vi "test_DependencyList_FilterByMatchingString.vi"() -> (3 "Pass?":bool)   [LabVIEW 2020, in "Tests.DependencyInspection.lvlib"]
uses:
  Tests.DependencyInspection.lvlib
  CDependencyList/CDependencyList.lvclass
  ItemInfo.ctl
  CItemMatch/CItemMatch.lvclass
  CItemMatch/TypeDefs/Field.ctl
  CItemMatch/TypeDefs/ComparisonType.ctl
  CDependencyList/ListGenerationOptions.ctl
panel:
  out "Array":string[](array[string])
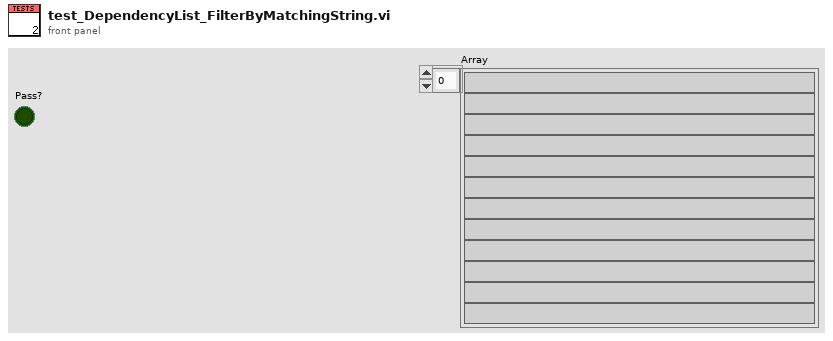
[diagram p1: front panel]
types:
  T1 = typedef "Tests.DependencyInspection.lvlib/ItemInfo.ctl" = cluster{"path":path, "delimited name":string}
  T2 = typedef "DependencyInspection.lvlib/CItemMatch.lvclass/ComparisonType.ctl" = enum16{"None", "Ends with", "Equals", "Not equal", "Starts with", "Contains", "Matches pattern"}
  T3 = typedef "DependencyInspection.lvlib/CItemMatch.lvclass/Field.ctl" = enum16{"Name", "Qualified name", "Path"}
  T4 = typedef "DependencyInspection.lvlib/CDependencyList.lvclass/ListGenerationOptions.ctl" = cluster{"exclude external?":bool, "exclude instances?":bool, "separate tests?":bool, "Root Path":path}
  T5 = typedef "NI_FileType.lvlib/LVFileType.ctl" = enum32{"Invalid file", "Unknown type", "Instrument", "Control", "Polymorphic VI", "Project", "Library", "LVClass", "XControl", "XNode", "Shared library", ".NET assembly", "ActiveX interface", "CIN", "Run-time menu", "Palette menu", "Help file", "LLB", "XNode Edit Dependency", "Class Private Data Control", "Statechart", "MathScript .m file", "Ladder Diagram", "LVLibp", "XNode Build Dependency"}
  T6 = cluster{"path":path, "delimited name":string, "type":T5, "iState":u32, "iStyle":u16, "wStyle":u16, "buttons":u16, "viflags":u32, "viflags2":u32, "links":u32[]}[]
  T7 = typedef "DependencyInspection.lvlib/CDependencyList.lvclass/DependencyList.ctl" = map{string, refnum<class "ILabVIEWItem.lvclass">}
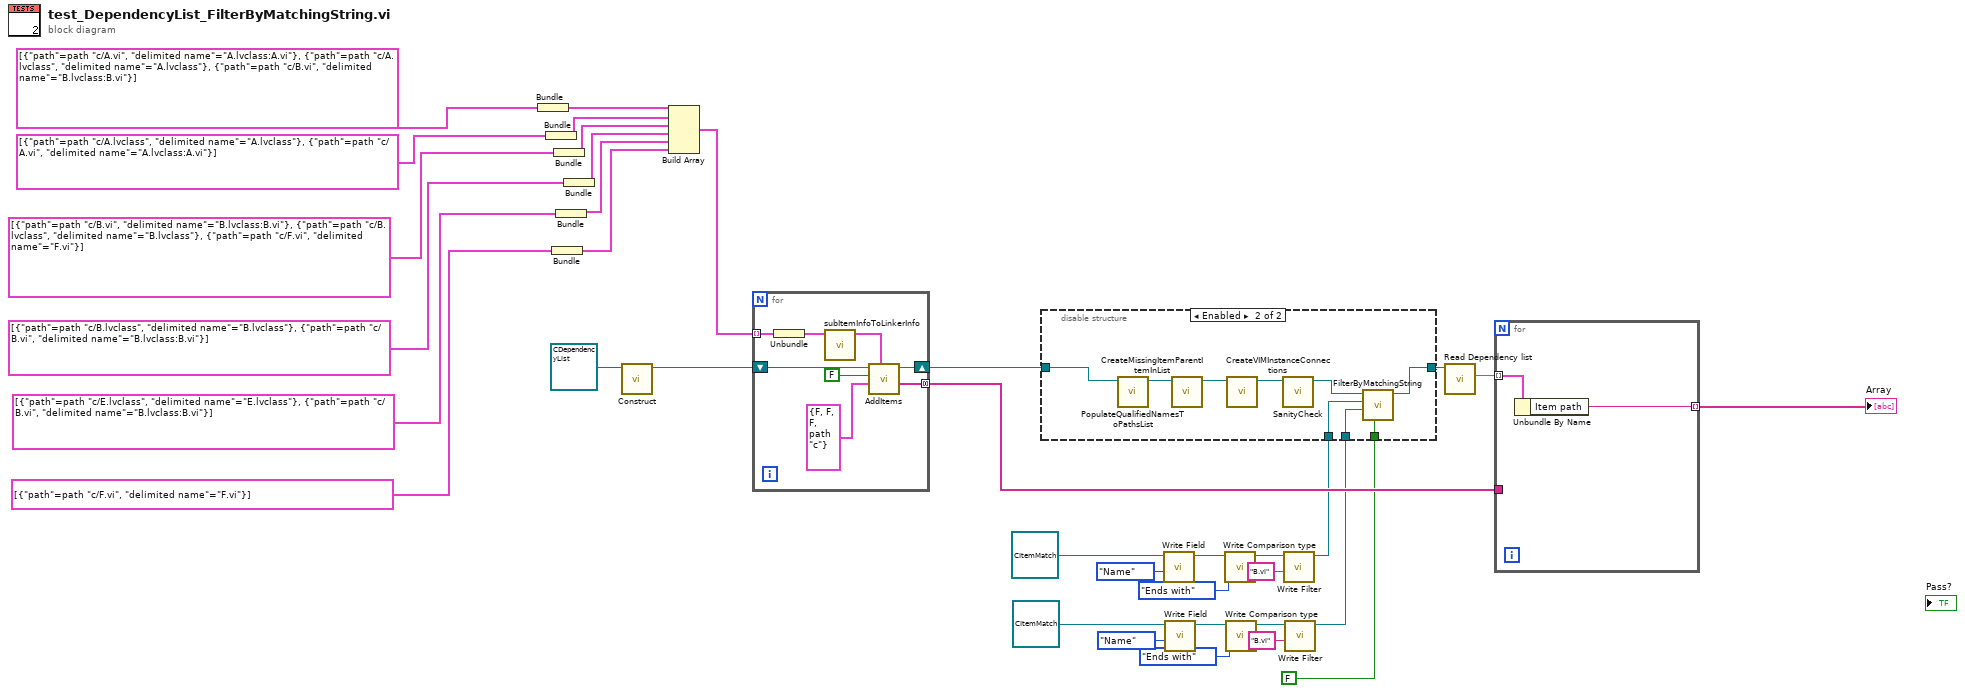
[diagram p0: block diagram]
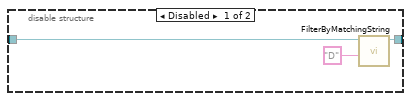
[diagram p2: hidden frame]
diagram:
  n1 = Bundle(T1[] [{"path"=path "c:/A.vi", "delimited name"="A.lvclass:A.vi"}, {"path"=path "c:/A.lvclass", "delimited name"="A.lvclass"}, {"path"=path "c:/B.vi", "delimited name"="B.lvclass:B.vi"}]) -> (w24:cluster{T1[]})  [unwired: 1 in]
  n2 = Bundle(T1[] [{"path"=path "c:/A.lvclass", "delimited name"="A.lvclass"}, {"path"=path "c:/A.vi", "delimited name"="A.lvclass:A.vi"}]) -> (w23:cluster{T1[]})  [unwired: 1 in]
  n3 = Bundle(T1[] [{"path"=path "c:/F.vi", "delimited name"="F.vi"}]) -> (w2:cluster{T1[]})  [unwired: 1 in]
  n4 = Bundle(T1[] [{"path"=path "c:/B.vi", "delimited name"="B.lvclass:B.vi"}, {"path"=path "c:/B.lvclass", "delimited name"="B.lvclass"}, {"path"=path "c:/F.vi", "delimited name"="F.vi"}]) -> (w22:cluster{T1[]})  [unwired: 1 in]
  n5 = Bundle(T1[] [{"path"=path "c:/E.lvclass", "delimited name"="E.lvclass"}, {"path"=path "c:/B.vi", "delimited name"="B.lvclass:B.vi"}]) -> (w18:cluster{T1[]})  [unwired: 1 in]
  n6 = Bundle(T1[] [{"path"=path "c:/B.lvclass", "delimited name"="B.lvclass"}, {"path"=path "c:/B.vi", "delimited name"="B.lvclass:B.vi"}]) -> (w21:cluster{T1[]})  [unwired: 1 in]
  n7 = call-dynamic "Construct.vi"("CDependencyList in"=refnum<class "CDependencyList.lvclass"> refnum) -> ("CDependencyList out"=w34:refnum<class "CDependencyList.lvclass">)  [unwired: 9 in, 1 out]
  n8 = Build Array(w24, w23, w22, w21, w18, w2) -> (w20:cluster{T1[]}[])
  n9 = for {
    tunnel: [w38] -> w29 mode=concatenating
    shift-right: [w42] -> w33
    shift-left: w34 -> [w43]
    tunnel: w20 -> [w37] mode=indexing
    n10 = Unbundle(w37) -> (w36:T1[])
    n11 = call "subItemInfoToLinkerInfo.vi"("Item info[]"=w36) -> ("Linker.Read Info From File"=w41:T6)  [unwired: 10 in]
    n12 = call-dynamic "AddItems.vi"("Linker.Read Info From File"=w41, "Settings"=T4 {"exclude external?"=FALSE, "exclude instances?"=FALSE, "separate tests?"=FALSE, "Root Path"=path "c:/"}, "Shallow deps?"=FALSE, "CDependencyList in"=w43) -> ("Debug messages"=w38:string[], "CDependencyList out"=w42:refnum<class "CDependencyList.lvclass">)  [unwired: 4 in, 2 out]
  }
  n13 = call-dynamic "Write Field.vi"("Field"=Field."Name", "CItemMatch in"=refnum<class "CItemMatch.lvclass"> refnum ("Target filter")) -> ("CItemMatch out"=w16:refnum<class "CItemMatch.lvclass">)  [unwired: 9 in]
  n14 = call-dynamic "Write Field.vi"("Field"=Field."Name", "CItemMatch in"=refnum<class "CItemMatch.lvclass"> refnum ("Target filter")) -> ("CItemMatch out"=w12:refnum<class "CItemMatch.lvclass">)  [unwired: 9 in]
  n15 = call-dynamic "Write Comparison type.vi"("Comparison type"=ComparisonType."Ends with", "CItemMatch in"=w16) -> ("CItemMatch out"=w15:refnum<class "CItemMatch.lvclass">)  [unwired: 9 in]
  n16 = call-dynamic "Write Comparison type.vi"("Comparison type"=ComparisonType."Ends with", "CItemMatch in"=w12) -> ("CItemMatch out"=w13:refnum<class "CItemMatch.lvclass">)  [unwired: 9 in]
  n17 = call-dynamic "Write Filter.vi"("Filter"="B.vi", "CItemMatch in"=w15) -> ("CItemMatch out"=w14:refnum<class "CItemMatch.lvclass">)  [unwired: 9 in]
  n18 = call-dynamic "Write Filter.vi"("Filter"="B.vi", "CItemMatch in"=w13) -> ("CItemMatch out"=w10:refnum<class "CItemMatch.lvclass">)  [unwired: 9 in]
  n19 = disable-structure shown="Enabled" {
    disable-tunnel: w33 -> [w44 w52]
    disable-tunnel: [w45 w50] -> w32
    disable-tunnel: w14 -> [_ w49]
    disable-tunnel: w10 -> [_ w48]
    disable-tunnel: FALSE ("AND Condition?") -> [_ w47]
    frame Disabled {
      n20 = call-dynamic "FilterByMatchingString.vi"("Target filter"="D", "CDependencyList in"=w44) -> ("CDependencyList out"=w45:refnum<class "CDependencyList.lvclass">)  [unwired: 8 in, 1 out]
    }
    frame Enabled {
      n21 = call-dynamic "PopulateQualifiedNamesToPathsList.vi"("CDependencyList in"=w52) -> ("CDependencyList out"=w53:refnum<class "CDependencyList.lvclass">)  [unwired: 9 in, 1 out]
      n22 = call-dynamic "CreateMissingItemParentItemInList.vi"("CDependencyList in"=w53) -> ("CDependencyList out"=w55:refnum<class "CDependencyList.lvclass">)  [unwired: 9 in, 1 out]
      n23 = call-dynamic "CreateVIMInstanceConnections.vi"("CDependencyList in"=w55) -> ("CDependencyList out"=w54:refnum<class "CDependencyList.lvclass">)  [unwired: 9 in, 1 out]
      n24 = call-dynamic "SanityCheck.vi"("CDependencyList in"=w54) -> ("CDependencyList out"=w51:refnum<class "CDependencyList.lvclass">)  [unwired: 8 in, 2 out]
      n25 = call-dynamic "FilterByMatchingString.vi"("AND Condition?"=w47, "Target filter"=w48, "Source filter"=w49, "CDependencyList in"=w51) -> ("CDependencyList out"=w50:refnum<class "CDependencyList.lvclass">)  [unwired: 6 in, 1 out]
    }
  }
  n26 = call-dynamic "Read Dependency list.vi"("CDependencyList in"=w32) -> ("Dependency List"=w31:T7)  [unwired: 9 in, 1 out]
  n27 = for {
    tunnel: w31 -> [w57] mode=indexing
    tunnel: [w56] -> w30 mode=indexing
    tunnel: w29 -> [_]
    n28 = Unbundle By Name(w57) -> ("Item path"=w56:string)
  }
  "Array" <- w30
